vi "Parse_procotol.vi"(8 "error in (no error)":errorcluster caption="错误输入（无错误）", 9 "DATA":string, 10 "ID":T1, 11 "Procotol_class 输入":refnum<class "Procotol_class.lvclass">) -> (0 "error out":errorcluster caption="错误输出", 1 "Mean":string[](array[string]), 2 "ARR_numb":string[](array[string]), 3 "Procotol_class 输出":refnum<class "Procotol_class.lvclass">, 4 "Valid/Matched?":bool[](array[boolean]))   [LabVIEW 2025, in "Procotol_class.lvclass"]
uses:
  Procotol_class.lvclass
  ID_arr.ctl
  Procotol_class.lvclass/Procotol_class.ctl
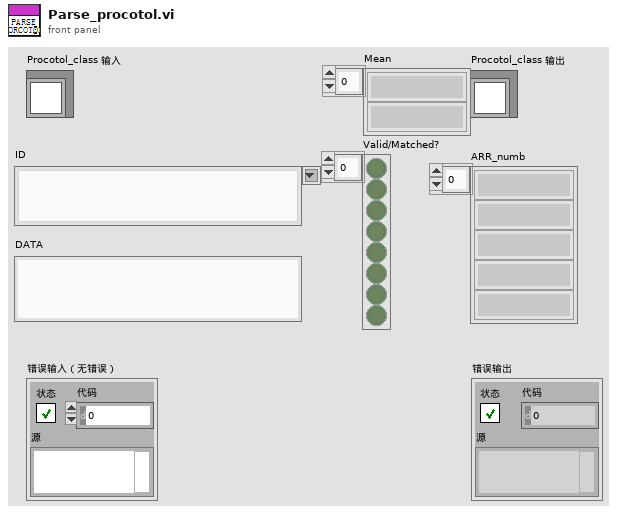
[diagram p1: front panel]
types:
  T1 = typedef "Procotol_class.lvclass/ID_arr.ctl" = string
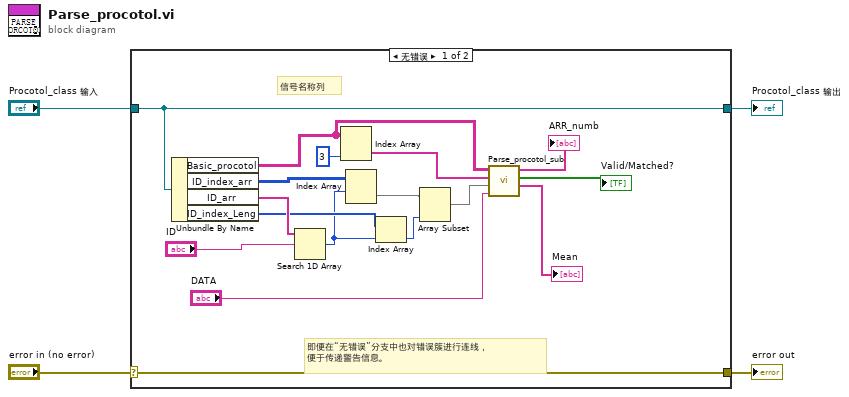
[diagram p0: block diagram]
diagram:
  n1 = case shown="无错误" "error in (no error)" {
    selector: "error in (no error)" -> [w21 w23]
    tunnel: [w21 w23] -> w3
    tunnel: [w20 w22] -> w1
    tunnel: "Procotol_class 输入" -> [w20 w22]
    frame No Error {
      # "信号名称列"
      # "即便在“无错误”分支中也对错误簇进行连线，\n便于传递警告信息。"
      n2 = Unbundle By Name(w20) -> ("Basic_procotol"=w15:string[][], "ID_index_arr"=w19:i32[][], "ID_arr"=w18:string[], "ID_index_Leng"=w7:i32[])
      n3 = Search 1D Array(1D array=w18, element="ID") -> (index of element=w6:i32)  [unwired: 1 in]
      n4 = Index Array(array=w15, index (col)=3 ("禁用的索引 (列)")) -> (element=w14:string[])  [unwired: 1 in]
      n5 = Index Array(array=w19, index (row)=w6) -> (element=w9:i32[])  [unwired: 1 in]
      n6 = Index Array(array=w7, index=w6) -> (element=w5:i32)
      n7 = Array Subset(array=w9, length=w5) -> (w8:i32[])  [unwired: 1 in]
      n8 = call "Parse_procotol_sub.vi"("Frame"="DATA", "ID_index"=w8, "Name_signal"=w14, "Procotol"=w15) -> ("Mean"=→"Mean":string[], "Valid/Matched?"=→"Valid/Matched?":bool[], "ARR_numb"=→"ARR_numb":string[])  [unwired: 5 in]
    }
    frame Error {
    }
  }
  "error out" <- w3
  "Procotol_class 输出" <- w1
